vi "On Start.vi"(8 "error in":errorcluster, 9 "Channel Settings":T1[](array[typedef]), 10 "Mode":T4, 11 "file path":path) -> (0 "error out":errorcluster, 3 "file reference":refnum<file>)   [LabVIEW 2021, in "Logging.lvlib"]
doc: "Open the data log file in 'file path'. If 'Mode' is 'Overwrite' or 'Create New', create an empty file and write a header with columns for timestamps and channel names according to 'Channel Settings'. Otherwise if 'Mode' is 'Append', open the data log file and seek to its end."
uses:
  Logging.lvlib
  Logging Mode.ctl
  Acquisition/Channel Settings.ctl
  Acquisition/IO Device.ctl
  Acquisition/Sensor Type.ctl
  Acquisition/Acquisition.lvlib
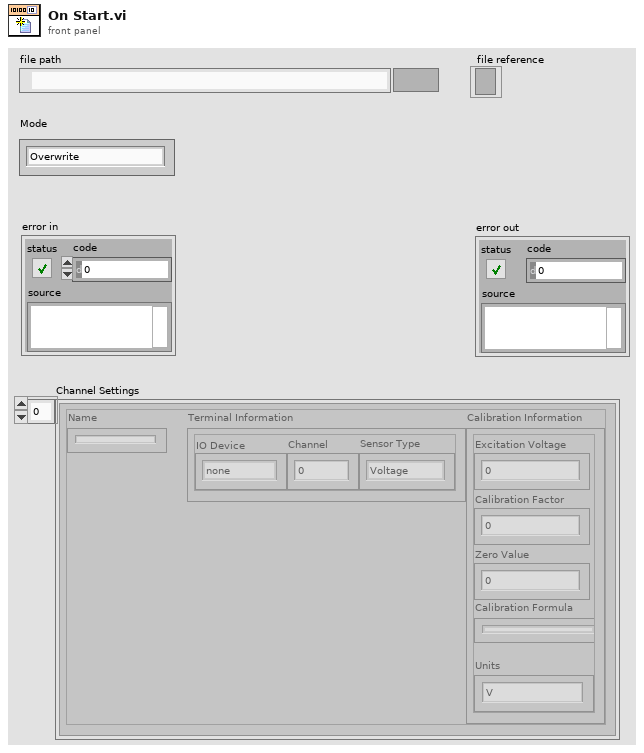
[diagram p1: front panel]
types:
  T1 = typedef "Acquisition.lvlib/Channel Settings.ctl" = cluster{"Name":string, "Terminal Information":cluster{"IO Device":T2, "Channel":i32, "Sensor Type":T3}, "Calibration Information":cluster{"Excitation Voltage":dbl, "Calibration Factor":dbl, "Zero Value":dbl, "Calibration Formula":string, "Units":string}}
  T2 = typedef "Acquisition.lvlib/IO Device.ctl" = enum16{"none", "9219", "9401"}
  T3 = typedef "Acquisition.lvlib/Sensor Type.ctl" = enum16{"Voltage", "Load", "Pressure", "Encoder"}
  T4 = typedef "Logging.lvlib/Logging Mode.ctl" = enum16{"Overwrite", "Append", "Create New"}
  T5 = enum16{"open", "replace", "create", "open or create", "replace or create", "replace or create with confirmation"}
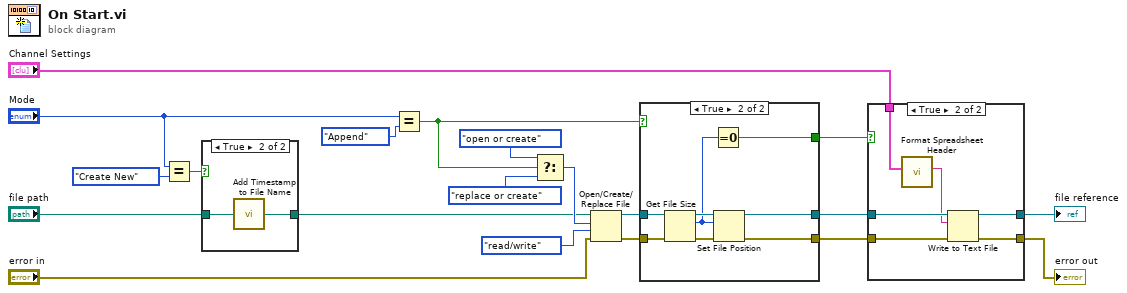
[diagram p0: block diagram]
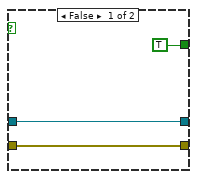
[diagram p4: hidden frame]
diagram:
  n1 = Equal?(x="Mode", y=Logging_Mode."Create New" ("Mode")) -> (x = y?=w1:bool)
  n2 = case shown="True" w1 {
    tunnel: "file path" -> [w21 w23]
    tunnel: [w21 w22] -> w4
    frame False {
    }
    frame True {
      n3 = call "Add Timestamp to File Name.vi"("base path"=w23) -> ("timestamped path"=w22:path)
    }
  }
  n4 = Equal?(x="Mode", y=Logging_Mode."Append" ("Mode")) -> (x = y?=w6:bool)
  n5 = Select(t=T5."open or create" ("operation (0:open)"), s=w6, f=T5."replace or create" ("operation (0:open)")) -> (s? t:f=w15:T5)
  n6 = Open/Create/Replace File(file path (use dialog)=w4, error in="error in", operation (0:open)=w15, access (0:read/write)=enum16{"read/write", "read-only", "write-only"}."read/write") -> (refnum out=w13:refnum<file>, error out=w12:errorcluster)  [unwired: 2 in, 1 out]
  n7 = case shown="True" w6 {
    tunnel: w13 -> [w25 w33]
    tunnel: w12 -> [w26 w32]
    tunnel: [w26 w30] -> w9
    tunnel: [w25 w29] -> w10
    tunnel: [TRUE w28] -> w11
    frame False {
    }
    frame True {
      n8 = Get File Size(file=w33, error in=w32) -> (refnum out=w34:refnum<file>, size (in bytes)=w27:i64, 0:w31:errorcluster)
      n9 = Equal To 0?(x=w27) -> (x = 0?=w28:bool)
      n10 = Set File Position(offset (in bytes) (0)=w27, refnum=w34, error in=w31) -> (refnum out=w29:refnum<file>, error out=w30:errorcluster)  [unwired: 1 in]
    }
  }
  n11 = case shown="True" w11 {
    tunnel: [w35 w42] -> w18
    tunnel: [w36 w41] -> w17
    tunnel: w10 -> [w36 w40]
    tunnel: w9 -> [w35 w39]
    tunnel: "Channel Settings" -> [_ w37]
    frame False {
    }
    frame True {
      n12 = call "Format Spreadsheet Header.vi"("Channel Settings"=w37) -> ("Log file header"=w38:string)  [unwired: 10 in]
      n13 = Write to Text File(file (use dialog)=w40, text=w38, error in=w39) -> (refnum out=w41:refnum<file>, error out=w42:errorcluster)  [unwired: 1 in, 1 out]
    }
  }
  "file reference" <- w17
  "error out" <- w18
